vi "Channel Name.vi"(8 "error in (no error)":errorcluster, 11 "Scale in":refnum<class "Scale Config.lvclass">) -> (0 "error out":errorcluster, 1 "Is Channel":bool, 2 "Channel Name":string, 3 "Scale out":refnum<class "Scale Config.lvclass">)   [LabVIEW 2020, in "VolatusConfig.lvlib" / "Scale Config.lvclass"]
uses:
  Scale Config.lvclass
  Scale Config.lvclass/Scale Config.ctl
  VolatusConfigElement/VolatusConfigElement.lvclass
  VolatusConfig.lvlib
  Meta Type.ctl
  lv-cdm/CDM-Config/Config Element/Config Element.lvclass
  C:/dev/lv20CE/relink/lv-volatus/VolatusConfig/VolatusConfigElement/VolatusConfigElement.lvclass
  C:/dev/lv20CE/relink/lv-volatus/VolatusConfig/Scale/Scale Config.lvclass
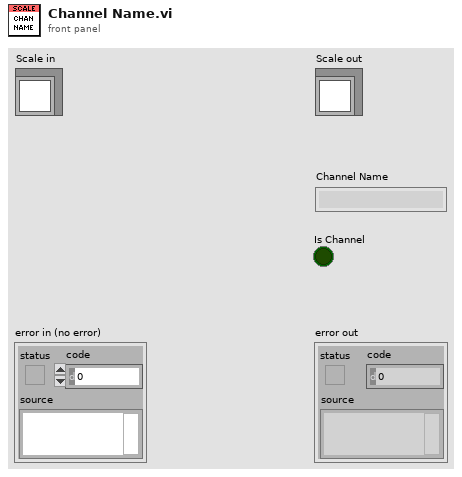
[diagram p1: front panel]
types:
  T1 = typedef "VolatusConfig.lvlib/Meta Type.ctl" = enum16{"UNKNOWN", "VL_System", "VL_Cluster", "VL_Node", "VL_Task", "VL_Group", "VL_Channel", "VL_Task_List", "VL_Scaling", "VL_Sensor", "VL_Sensor_List", "VL_Scale"}
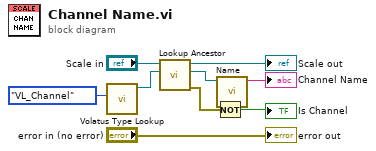
[diagram p0: block diagram]
diagram:
  n1 = call "Volatus Type Lookup.vi"("Meta Type"=Meta_Type."VL_Channel") -> ("Config Lookup out"=w5:refnum<class "Config Lookup.lvclass">)  [unwired: 9 in, 1 out]
  n2 = call "Lookup Ancestor.vi"("Lookup"=w5, "VolatusConfigElement in"="Scale in") -> ("error out"=w2:errorcluster, "Ancestor"=w4:refnum<class "Config Element.lvclass">, "VolatusConfigElement out"=→"Scale out":refnum<class "Scale Config.lvclass">)  [unwired: 7 in]
  n3 = Not(x=w2) -> (.not. x?=→"Is Channel":bool)
  n4 = call "Name.vi"("Config Element in"=w4) -> ("Name"=→"Channel Name":string)  [unwired: 9 in, 1 out]
  "error out" <- "error in (no error)"
